vi "str to uint8array.vi"(2 "String":string) -> (6 "uint8 array":u8[](array[numeric]))   [LabVIEW 2014, in "OPCUA XML(dev).lvlib"]
uses:
  OPCUA XML(dev).lvlib
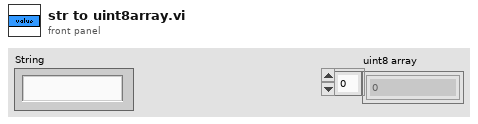
[diagram p1: front panel]
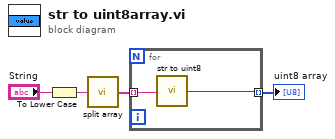
[diagram p0: block diagram]
diagram:
  n1 = To Lower Case(string="String") -> (all lower case string=w3:string)
  n2 = call "split array.vi"("string"=w3) -> ("split arr"=w2:string[])  [unwired: 8 in]
  n3 = for {
    tunnel: w2 -> [w6] mode=indexing
    tunnel: [w5] -> w1 mode=indexing
    n4 = call "str to uint8.vi"("String"=w6) -> ("uint8"=w5:u8)  [unwired: 6 in]
  }
  "uint8 array" <- w1
